vi "Register Test.vi"(8 "error in (no error)":errorcluster, 9 "VI Call Chain":string[](array[string]), 10 "Test Label":string, 11 "Assert Factory in":refnum<class "Test Assert Factory.lvclass">) -> (0 "error out":errorcluster, 1 "Caller ID":string, 2 "Test ID":string, 3 "Assert Factory out":refnum<class "Test Assert Factory.lvclass">, 4 "Tests to Register":T1[](array[typedef]))   [LabVIEW 2020, in "Caraya.lvlib" / "Test Assert Factory.lvclass"]
doc: "Registers a Test VI with the Assert Factory"
uses:
  Test Assert Factory.lvclass
  Test Storage -- cluster.ctl
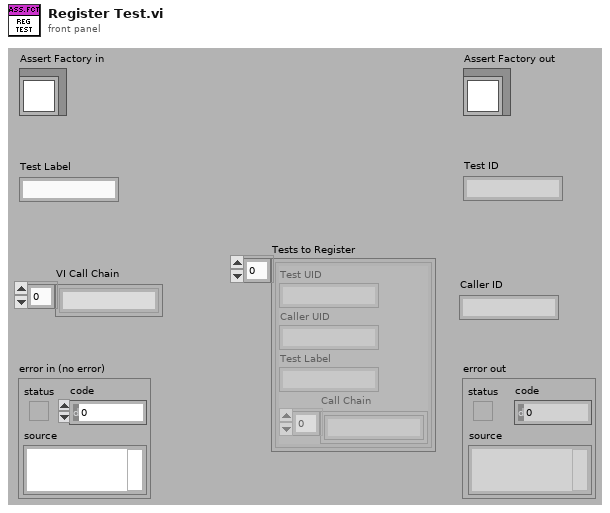
[diagram p1: front panel]
types:
  T1 = typedef "Caraya.lvlib/Test Assert Factory.lvclass/Test Storage -- cluster.ctl" = cluster{"Test UID":string, "Caller UID":string, "Test Label":string, "Call Chain":string[]}
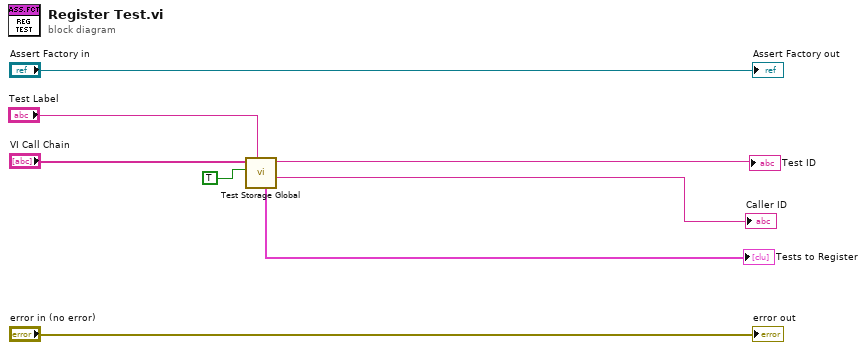
[diagram p0: block diagram]
diagram:
  n1 = call "Test Storage Global.vi"("Test Label"="Test Label", "Set (F)"=TRUE, "VI Call Chain"="VI Call Chain") -> ("Caller ID"=→"Caller ID":string, "Unique Test ID"=→"Test ID":string, "Tests to Register"=→"Tests to Register":T1[])  [unwired: 5 in, 1 out]
  "error out" <- "error in (no error)"
  "Assert Factory out" <- "Assert Factory in"
